vi "IRregulatetest.vi"(8 "error in (no error)":errorcluster, 9 "Enum":T2(ring), 10 "左後距離":dbl=1.265, 11 "右後距離":dbl=1.245) -> (0 "error out":errorcluster)   [LabVIEW 2019]
uses:
  <vilib>/Platform/TimedLoop/XDataNode/timing_clust.ctl
  <vilib>/Platform/TimedLoop/XDataNode/nitl_modes.ctl
  <vilib>/Platform/TimedLoop/XDataNode/wakeup.ctl
  <vilib>/platform/TimedLoop/XDataNode/XDataNode.xnode
  <vilib>/Platform/TimedLoop/XDataNode/XDNodeRunTimeDep.lvlib
panel:
  out "x .or. y?":bool
  out "Numeric":i32
  in  "左前距離":dbl=1.3
  in  "右前距離":dbl=1.3
  out "紅外線數值":T1
  out "Array":dbl[](array[numeric])
  in  "stop":bool
  out "output":dbl[](array[numeric])=[100.0, -100.0]
  out "誤差":dbl[](array[numeric])=[10401.0, -10400.0]
  in  "右邊距離":dbl
  # "4"
  # "1.28\n1.3"
  # "1.245\n1.265"
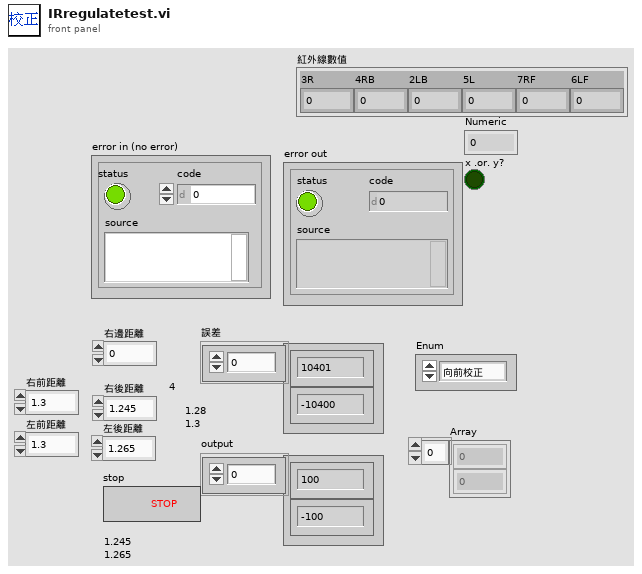
[diagram p1: front panel]
types:
  T1 = cluster{"7RF":dbl, "3R":dbl, "4RB":dbl, "5L":dbl, "6LF":dbl, "2LB":dbl}
  T2 = enum16{"向前校正", "向後校正", "右後校正", "右前校正", "左前校正", "左後校正", ""}
  T3 = typedef "AI.lvlib/AI Reference.ctl" = cluster{"myRIO Reference":T4, "AI Channels List":T8, "AI Scaling Constants List":T10}
  T4 = typedef "myRIO Generic Hardware Reference.ctl" = cluster{"myRIO Model":T5, "myRIO Hardware Reference":T6}
  T5 = typedef "Hardware Version Enum.ctl" = enum16{"Unknown", "myRIO-1900", "myRIO-1950", "roboRIO", "NI ELVIS RIO CM", "ELVIS III"}
  T6 = typedef "myRIO v1.0 Reference.ctl" = cluster{"Generic FPGA Reference":T7, "Allow multiple opens":bool}
  T7 = typedef "Generic FPGA Reference.ctl" = refnum<k20>
  T8 = typedef "AI Channels List.ctl" = T9[]
  T9 = typedef "AI Channels Enum.ctl" = enum16{"Not Connected", "AudioIn/Left", "AudioIn/Right", "C/AI0", "C/AI1", "A/AI0", "A/AI1", "A/AI2", "A/AI3", "A/AI4", "A/AI5", "A/AI6", "A/AI7", "B/AI0", "B/AI1", "B/AI2", "B/AI3", "B/AI4", "B/AI5", "B/AI6", "B/AI7", "AI/AI0", "AI/AI1", "AI/AI2", "AI/AI3", "A/AI0 (DIFF)", "A/AI1 (DIFF)", "A/AI2 (DIFF)", "A/AI3 (DIFF)", "B/AI0 (DIFF)", "B/AI1 (DIFF)", "B/AI2 (DIFF)", "B/AI3 (DIFF)"}
  T10 = typedef "Analog Scaling Constants List.ctl" = T11[]
  T11 = typedef "Analog Scaling Constants.ctl" = cluster{"LSB Weight (Volts)":dbl, "Offset (Volts)":dbl, "Signed?":bool}
  T12 = typedef "XDNodeRunTimeDep.lvlib/timing_clust.ctl" = cluster{"Expected End [f-1]":u64, "Actual End [f-1]":u64, "Finished Late? [f-1]":bool, "Expected End [i-1]":u64, "Actual End [i-1]":u64, "Finished Late? [i-1]":bool, "Expected Start [i]":u64, "Actual Start [i]":u64, "Expected Start [f]":u64, "Actual Start [f]":u64, "Source Name":string, "Structure Name":string, "Period":i64, "Deadline":i64, "Offset":i64, "Start":i64, "Priority":i32, "Timeout":i32, "Mode":T13, "Wakeup Reason":T14, "Error":errorcluster, "Source Type":string, "Secondary Source Type":string, "Global End Time":u64, "Global Start Time":u64, "Frame Duration":u64, "Iteration Duration":u64, "Assigned CPU":i32, "I/O Scan Engine Mode":u32}
  T13 = typedef "XDNodeRunTimeDep.lvlib/nitl_modes.ctl" = enum32{"No Change", "Process missed periods, maintain original phase", "Discard missed periods, maintain original phase", "Process missed periods, ignore original phase", "Discard missed periods, ignore original phase"}
  T14 = typedef "XDNodeRunTimeDep.lvlib/wakeup.ctl" = enum32{"Normal", "Aborted", "Asynchronous wakeup", "Timing source error", "Timed loop error", "Timeout"}
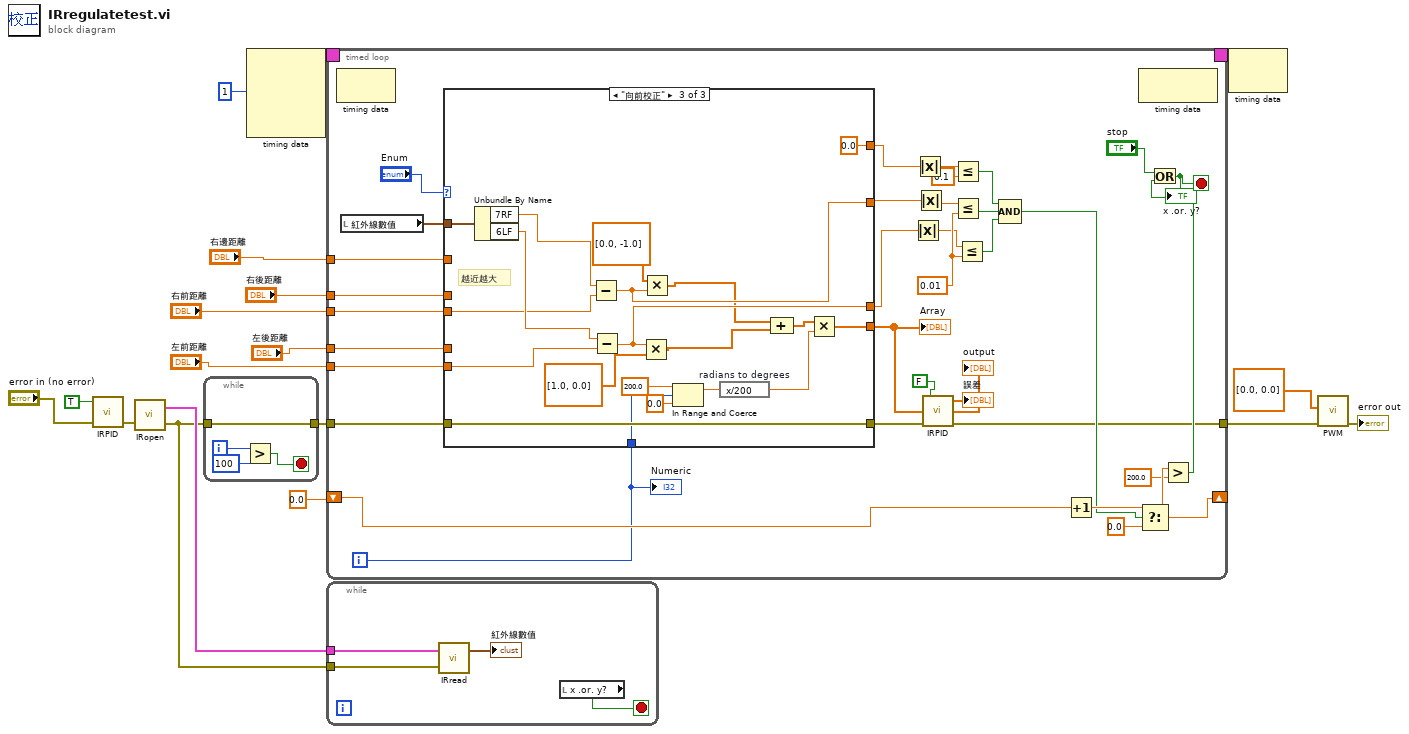
[diagram p0: block diagram]
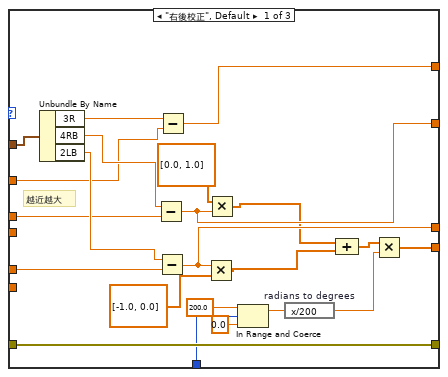
[diagram p2: hidden frame]
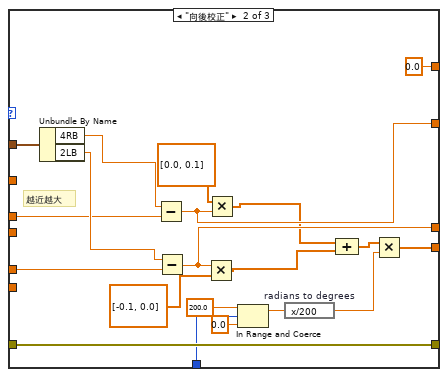
[diagram p3: hidden frame]
diagram:
  n1 = call "IRPID.vi"("error in (no error)"="error in (no error)", "Reset"=TRUE ("s")) -> ("error out"=w5:errorcluster)  [unwired: 1 in, 2 out]
  n2 = call "IRopen.vi"("error in (no error)"=w5) -> ("error out"=w2:errorcluster, "AI Ref Out"=w3:T3)  [unwired: 1 in]
  n3 = while {
    tunnel: w2 -> [w22]
    tunnel: [w22] -> w1
    i -> [w20]
    stop <- w21 stop-if-true
    n4 = Greater?(x=w20, y=100) -> (0:w21:bool)
  }
  n5 = node-c288(i64 1 ("Period")) -> (w18:T12)  [unwired: 3 in]
  n6 = timed-loop {
    timing: w18 -> [_]
    timing-out: [_] -> w17
    tunnel: w1 -> [w39]
    shift-right: [w51] -> _
    shift-left: 0.0 -> [w52]
    tunnel: "右邊距離" -> [w48]
    tunnel: "右後距離" -> [w47]
    tunnel: "左後距離" -> [w46]
    tunnel: "右前距離" -> [w45]
    tunnel: "左前距離" -> [w44]
    tunnel: [w40] -> w7
    i -> [w43]
    stop <- w55 stop-if-true
    w32 = 0.01 ("y")
    n7 = node-c288() -> ()  [unwired: 1 in, 1 out]
    n8 = local read "紅外線數值"() -> (w38:T1)
    n9 = case shown="\"向前校正\"" "Enum" {
      tunnel: [w78 w98 w118] -> w40
      tunnel: w39 -> [w78 w98 w118]
      tunnel: [w66 w87 w107] -> w26
      tunnel: w43 -> [w71 w92 w112]
      tunnel: [w65 0.0 0.0] -> w23
      tunnel: [w64 w86 w106] -> w24
      tunnel: [w63 w85 w105] -> w25
      tunnel: w48 -> [w60 _ _]
      tunnel: w47 -> [w59 w82 _]
      tunnel: w46 -> [w58 w81 _]
      tunnel: w45 -> [_ _ w101]
      tunnel: w44 -> [_ _ w100]
      tunnel: w38 -> [w57 w79 w99]
      frame "右後校正", Default {
        # "越近越大"
        n10 = Unbundle By Name(w57) -> ("3R"=w77:dbl, "4RB"=w76:dbl, "2LB"=w75:dbl)
        n11 = Subtract(x=w76, y=w59) -> (x-y=w64:dbl)
        n12 = Subtract(x=w75, y=w58) -> (x-y=w63:dbl)
        n13 = Subtract(x=w77, y=w60) -> (x-y=w65:dbl)
        n14 = Multiply(x=w63, y=dbl[] [-1.0, 0.0] ("x")) -> (x*y=w62:dbl[])
        n15 = Multiply(x=dbl[] [0.0, 1.0], y=w64) -> (x*y=w61:dbl[])
        n16 = In Range and Coerce(upper limit=200.0, x=w71, lower limit=0.0) -> (coerced(x)=w68:dbl)  [unwired: 1 out]
        n17 = expression code="x/200" "radians to degrees"(w68) -> (w67:dbl)
        n18 = Compound Arithmetic op=ADD(w61, w62) -> (w72:dbl[])
        n19 = Multiply(x=w72, y=w67) -> (x*y=w66:dbl[])
      }
      frame "向後校正" {
        # "越近越大"
        n20 = Unbundle By Name(w79) -> ("4RB"=w97:dbl, "2LB"=w96:dbl)
        n21 = Subtract(x=w97, y=w82) -> (x-y=w86:dbl)
        n22 = Subtract(x=w96, y=w81) -> (x-y=w85:dbl)
        n23 = Multiply(x=w85, y=dbl[] [-0.1, 0.0] ("x")) -> (x*y=w84:dbl[])
        n24 = Multiply(x=dbl[] [0.0, 0.1], y=w86) -> (x*y=w83:dbl[])
        n25 = In Range and Coerce(upper limit=200.0, x=w92, lower limit=0.0) -> (coerced(x)=w89:dbl)  [unwired: 1 out]
        n26 = expression code="x/200" "radians to degrees"(w89) -> (w88:dbl)
        n27 = Compound Arithmetic op=ADD(w83, w84) -> (w93:dbl[])
        n28 = Multiply(x=w93, y=w88) -> (x*y=w87:dbl[])
      }
      frame "向前校正" {
        # "越近越大"
        n29 = Unbundle By Name(w99) -> ("7RF"=w117:dbl, "6LF"=w116:dbl)
        n30 = Subtract(x=w117, y=w101) -> (x-y=w106:dbl)
        n31 = Subtract(x=w116, y=w100) -> (x-y=w105:dbl)
        n32 = Multiply(x=w105, y=dbl[] [1.0, 0.0] ("x")) -> (x*y=w104:dbl[])
        n33 = Multiply(x=dbl[] [0.0, -1.0], y=w106) -> (x*y=w103:dbl[])
        n34 = In Range and Coerce(upper limit=200.0, x=w112, lower limit=0.0) -> (coerced(x)=w109:dbl)  [unwired: 1 out]
        n35 = expression code="x/200" "radians to degrees"(w109) -> (w108:dbl)
        n36 = Compound Arithmetic op=ADD(w103, w104) -> (w113:dbl[])
        n37 = Multiply(x=w113, y=w108) -> (x*y=w107:dbl[])
      }
    }
    "Array" <- w26
    n38 = Absolute Value(x=w25) -> (abs(x)=w30:dbl)
    n39 = Absolute Value(x=w23) -> (abs(x)=w29:dbl)
    n40 = Absolute Value(x=w24) -> (abs(x)=w31:dbl)
    n41 = call "IRPID.vi"("目標"=w26, "Reset"=FALSE) -> ("output"=→"output":dbl[], "誤差"=→"誤差":dbl[])  [unwired: 1 in, 1 out]
    n42 = Less Or Equal?(x=w29, y=0.1) -> (x <= y?=w33:bool)
    n43 = Less Or Equal?(x=w31, y=w32) -> (x <= y?=w34:bool)
    n44 = Less Or Equal?(x=w30, y=w32) -> (x <= y?=w35:bool)
    n45 = Compound Arithmetic op=AND(w33, w34, w35) -> (w41:bool)
    n46 = Increment(x=w52) -> (x+1=w53:dbl)
    n47 = node-c288() -> ()  [unwired: 1 in, 1 out]
    n48 = Select(t=w53, s=w41, f=0.0) -> (s? t:f=w51:dbl)
    n49 = Greater?(x=w51, y=200.0) -> (0:w49:bool)
    n50 = Or(x="stop", y=w49) -> (x .or. y?=w55:bool)
    "x .or. y?" <- w55
    "Numeric" <- w43
  }
  n51 = while {
    tunnel: w2 -> [w123]
    tunnel: w3 -> [w122]
    stop <- w121 stop-if-true
    n52 = call "IRread.vi"("error in (no error)"=w123, "AI Ref In"=w122) -> ("紅外線數值"=→"紅外線數值":T1)  [unwired: 1 out]
    n53 = local read "x .or. y?"() -> (w121:bool)
  }
  n54 = node-c288(w17) -> ()  [unwired: 1 out]
  n55 = call "PWM.vi"("error in (no error)"=w7, "power"=dbl[] [0.0, 0.0]) -> ("error out"=→"error out":errorcluster)  [unwired: 9 in]
